vi "UMLEditor Main.vi"(1 "StartProject":string, 3 "StartTarget":string) -> ()   [LabVIEW 2020] (continued)
                        n993 = Unbundle By Name(w2758) -> ("height"=w2757:dbl, "width"=w2754:dbl)
                        n994 = Unbundle By Name(w2751) -> ("Scrolling"=w2732:i32)
                        n995 = Tick Count (ms)() -> (millisecond timer value=w2749:u32)
                        n996 = Equal To 0?(x=w2747) -> (x = 0?=w2746:bool)
                        n997 = Subtract(x=w2749, y=w2747) -> (x-y=w2745:u32)
                        n998 = feedback-in #1(w2732) -> ()
                        n999 = feedback #1(w2732) -> (w2733:i32)
                        n1000 = Select(t=u32 0, s=w2746, f=w2745) -> (s? t:f=w2744:u32)
                        n1001 = Subtract(x=w2732, y=w2733) -> (x-y=w2729:i32)
                        n1002 = Not Equal To 0?(x=w2732) -> (x != 0?=w2731:bool)
                        n1003 = Not Equal To 0?(x=w2729) -> (x != 0?=w2730:bool)
                        n1004 = And(x=w2731, y=w2730) -> ()  [unwired: 1 out]
                        n1005 = case shown="0..750" w2744 {
                          tunnel: w2748 -> [w2764 w2765]
                          tunnel: [w2760 w2765] -> w2740
                          frame Default {
                            n1006 = property on="SearchString" class="Str"("Visible"=FALSE) -> ()  [unwired: 2 in, 2 out]
                            n1007 = local write "SearchString"("" ("SearchString")) -> ()
                            n1008 = Bundle By Name(cluster=w2764, "KeyPressTime"=u32 0) -> (w2760:T5)
                          }
                          frame 0..750 {
                          }
                        }
                        n1009 = case shown="False" FALSE {
                          tunnel: w2757 -> [_ w2910]
                          tunnel: w2756 -> [_ w2909]
                          tunnel: w2740 -> [w2777 w2908]
                          tunnel: [w2776 w2907] -> w2739
                          tunnel: [w2771 w2906] -> w2755
                          tunnel: w2752 -> [w2772 w2905]
                          tunnel: w2754 -> [_ w2904]
                          tunnel: w2750 -> [w2770 w2903]
                          tunnel: w2751 -> [w2779 _]
                          tunnel: w2734 -> [w2778 _]
                          tunnel: w2753 -> [w2775 _]
                          tunnel: w2742 -> [w2774 _]
                          tunnel: w2741 -> [w2773 _]
                          tunnel: [w2769 _] -> w2737
                          tunnel: [w2768 _] -> w2736
                          tunnel: w2735 -> [w2766 _]
                          tunnel: w2729 -> [_ w2901]
                          frame False {
                            n1010 = call <resource>:"UMLEditor_OnHotSpot.vi"("ZoomLevel"=w2766, "ObjectHotspots"=w2773, "Mouse Position"=w2774) -> ("Function"=w2768:T16, "HotSpotCursor"=w2769:bool, "Node"=w2767:refnum<class "AbstractNode.lvclass">)  [unwired: 5 in, 1 out]
                            n1011 = case shown="False" w2769 {
                              tunnel: w2779 -> [w2799 _]
                              tunnel: w2778 -> [w2796 _]
                              tunnel: w2777 -> [w2795 w2887]
                              tunnel: [w2794 w2886] -> w2776
                              tunnel: w2775 -> [w2787 _]
                              tunnel: w2772 -> [w2783 w2889]
                              tunnel: [w2783 w2888] -> w2771
                              tunnel: w2770 -> [_ _]
                              tunnel: w2768 -> [_ w2885]
                              tunnel: w2767 -> [_ w2884]
                              frame False {
                                n1012 = Unbundle By Name(w2799) -> ("Horizontal"=w2798:i32, "Vertical"=w2797:i32)
                                n1013 = property on="Project" class="Ring (strict)"() -> ("Strings []"=w2788:string[])  [unwired: 2 in, 2 out]
                                n1014 = Unbundle By Name(w2796) -> ("button 1"=w2784:bool)
                                n1015 = local read "Project"() -> (w2781:u16)
                                n1016 = Index Array(array=w2788, index=w2781) -> (element=w2782:string)
                                n1017 = Match Pattern(string=w2782, regular expression="^Untitled") -> (offset past match=w2791:i32)  [unwired: 4 out]
                                n1018 = case shown="False" w2784 {
                                tunnel: [_ w2802] -> w2785
                                frame False {
                                }
                                frame True {
                                n1019 = call <resource>:"UMLEditor_GetActiveWindow.vi"() -> ("Project Explorer"=w2802:bool)  [unwired: 1 in, 10 out]
                                }
                                }
                                n1020 = case shown="False" FALSE {
                                tunnel: w2798 -> [w2807 w2829]
                                tunnel: w2797 -> [w2806 w2828]
                                tunnel: w2785 -> [w2805 w2827]
                                tunnel: [w2804 w2826] -> w2793
                                tunnel: w2784 -> [w2803 w2825]
                                frame True {
                                n1021 = while {
                                shift-right: [w2813] -> _
                                shift-left: _ -> [w2812]
                                tunnel: w2807 -> [w2816]
                                tunnel: w2806 -> [w2815]
                                tunnel: w2805 -> [w2813]
                                tunnel: [w2814] -> w2804
                                tunnel: w2803 -> [w2810]
                                stop <- TRUE stop-if-true
                                # "Mouse inside VI"
                                n1022 = property class="VI"() -> ("Front Panel.WinBounds"=w2824:T52, "Front Panel.IsFrontmost"=w2808:bool)  [unwired: 2 in, 2 out]
                                n1023 = Not(x=w2808) -> (.not. x?=w2809:bool)
                                n1024 = Unbundle(w2824) -> ("Left"=w2823:i16, "Top"=w2820:i16, "Right"=w2822:i16, "Bottom"=w2821:i16)
                                n1025 = property on="DragAndDropPath" class="Path"("Visible"=w2809) -> ()  [unwired: 2 in, 2 out]
                                n1026 = In Range and Coerce(upper limit=w2822, x=w2816, lower limit=w2823) -> (In Range?=w2819:bool)  [unwired: 1 out]
                                n1027 = In Range and Coerce(upper limit=w2821, x=w2815, lower limit=w2820) -> (In Range?=w2818:bool)  [unwired: 1 out]
                                n1028 = And(x=w2819, y=w2818) -> (x .and. y?=w2811:bool)
                                n1029 = Compound Arithmetic op=AND(w2811, invert w2810, w2812) -> (w2814:bool)
                                }
                                }
                                frame False {
                                n1030 = while {
                                shift-right: [w2833] -> _
                                shift-left: _ -> [w2832]
                                tunnel: w2829 -> [w2836]
                                tunnel: w2828 -> [w2835]
                                tunnel: w2827 -> [w2833]
                                tunnel: [w2834] -> w2826
                                tunnel: w2825 -> [w2830]
                                stop <- TRUE stop-if-true
                                # "Mouse inside VI"
                                n1031 = property class="VI" props=["Front Panel.WinBounds", "Front Panel.IsFrontmost"]() -> ("Front Panel.WinBounds"=w2844:T52)  [unwired: 2 in, 3 out]
                                n1032 = Unbundle(w2844) -> ("Left"=w2843:i16, "Top"=w2840:i16, "Right"=w2842:i16, "Bottom"=w2841:i16)
                                n1033 = In Range and Coerce(upper limit=w2842, x=w2836, lower limit=w2843) -> (In Range?=w2839:bool)  [unwired: 1 out]
                                n1034 = In Range and Coerce(upper limit=w2841, x=w2835, lower limit=w2840) -> (In Range?=w2838:bool)  [unwired: 1 out]
                                n1035 = And(x=w2839, y=w2838) -> (x .and. y?=w2831:bool)
                                n1036 = Compound Arithmetic op=AND(w2831, invert w2830, w2832) -> (w2834:bool)
                                }
                                }
                                }
                                n1037 = while {
                                shift-right: [w2880] -> w2801
                                shift-left: _ -> [w2882]
                                stop <- TRUE stop-if-true
                                n1038 = Increment(x=w2882) -> (x+1=w2881:u8)
                                n1039 = To Unsigned Byte Integer(number=w2881) -> (unsigned 8bit integer=w2880:u8)
                                }
                                n1040 = Empty String/Path?(string/path=w2782) -> (empty?=w2800:bool)
                                n1041 = Greater Or Equal To 0?(x=w2791) -> (x >= 0?=w2790:bool)
                                n1042 = call <resource>:"UMLEditor_SetMouseCursor.vi"("error in (no error)"=w2783, "CursorType"=UMLEditor_Cursortype."Arrow") -> ()  [unwired: 8 in, 2 out]
                                n1043 = Or(x=w2800, y=w2790) -> (x .or. y?=w2789:bool)
                                n1044 = case shown="0" w2801 {
                                tunnel: w2789 -> [w2851 _ _ _]
                                tunnel: w2782 -> [w2850 _ _ _]
                                tunnel: w2787 -> [_ _ _ _]
                                tunnel: w2781 -> [w2849 _ _ _]
                                frame 0 {
                                n1045 = case shown="True" w2851 {
                                tunnel: w2850 -> [_ _]
                                tunnel: w2849 -> [_ w2855]
                                frame False {
                                }
                                frame True {
                                n1046 = call <resource>:"GDSProject_GetProjects.vi"("OpenProjectRef(True)"=FALSE) -> ("Projects"=w2858:string[], "error out"=w2861:errorcluster)  [unwired: 2 in, 15 out]
                                n1047 = Array Size(array=w2858) -> (size(s)=w2857:i32)
                                n1048 = Empty Array?(array=w2858) -> (empty?=w2862:bool)
                                n1049 = Decrement(x=w2857) -> (x-1=w2856:i32)
                                n1050 = Max & Min(x=w2856, y=w2855) -> (min(x,y)=w2854:i32)  [unwired: 1 out]
                                n1051 = Max & Min(x=w2854, y=0) -> (max(x,y)=w2852:i32)  [unwired: 1 out]
                                n1052 = Index Array(array=w2858, index=w2852) -> (element=w2860:string)
                                n1053 = property on="Project" class="Ring (strict)"("Strings []"=w2858, "Value"=w2852) -> ()  [unwired: 2 in, 2 out]
                                n1054 = case shown="False" w2862 {
                                tunnel: w2860 -> [w2868 _]
                                tunnel: w2861 -> [w2869 w2879]
                                tunnel: [w2866 w2878] -> _
                                frame False {
                                n1055 = call <resource>:"GetRelativePathOption.vi"() -> ("UseProjectFolderAsBasePath"=w2871:bool)  [unwired: 1 in, 18 out]
                                n1056 = call <resource>:"UMLEditor_TargetDialog.vi"("error in (no error)"=w2869, "Target"="My Computer" ("element"), "GetProjectRefByName"=w2868) -> ("error out"=w2866:errorcluster, "ProjectFolder"=w2867:path, "TargetIndex"=w2864:u16, "Targets"=w2865:string[])  [unwired: 4 in, 1 out]
                                n1057 = case shown="True" w2871 {
                                tunnel: w2867 -> [_ w2873]
                                tunnel: File_StoredPathesActions."Set Path" ("Method (Get Path)") -> [_ w2872]
                                frame False {
                                }
                                frame True {
                                n1058 = call <resource>:"File_ApplicationPaths.vi"("PathName"=UMLEditor_StoredPathes."ClassBasePath" ("UMLPathes"), "Path In"=w2873, "Method (Get Path)"=w2872) -> ()  [unwired: 1 in, 16 out]
                                }
                                }
                                n1059 = property on="Target" class="Ring (strict)"("Strings []"=w2865, "Value"=w2864) -> ()  [unwired: 2 in, 2 out]
                                }
                                frame True {
                                n1060 = call <resource>:"CommonVIs_UmlOpenVIRef.vi"("ProjectNameIn"="clear", "error in"=w2879) -> ("error out"=w2878:errorcluster)  [unwired: 2 in, 7 out]
                                n1061 = property on="Target" class="Ring (strict)"("Strings []"=string[] [], "Value"=u16 0 ("icon")) -> ()  [unwired: 2 in, 2 out]
                                }
                                }
                                }
                                }
                                }
                                frame 1 {
                                }
                                frame 2 {
                                }
                                frame Default {
                                }
                                }
                                n1062 = case shown="False" w2793 {
                                tunnel: w2795 -> [w2845 w2848]
                                tunnel: [w2845 w2847] -> w2794
                                frame False {
                                }
                                frame True {
                                n1063 = Bundle By Name(cluster=w2848, "state"=UMLEditor_statesType."AddNodeFromProjectTree") -> (w2847:T5)
                                }
                                }
                              }
                              frame True {
                                n1064 = case shown="Default" w2885 {
                                tunnel: w2889 -> [w2892 w2898]
                                tunnel: [w2890 w2899] -> w2888
                                tunnel: w2885 -> [w2893 _]
                                frame Default {
                                n1065 = case shown="\"SE\", \"NW\"" w2893 {
                                tunnel: [_ UMLEditor_Cursortype."NS" ("CursorType") UMLEditor_Cursortype."NESW" ("CursorType") UMLEditor_Cursortype."WE" ("CursorType") UMLEditor_Cursortype."NWSE" ("CursorType")] -> w2891
                                frame Default {
                                }
                                frame "N", "S" {
                                }
                                frame "NE", "SW" {
                                }
                                frame "E", "W" {
                                }
                                frame "SE", "NW" {
                                }
                                }
                                n1066 = call <resource>:"UMLEditor_SetMouseCursor.vi"("error in (no error)"=w2892, "CursorType"=w2891) -> ("error out"=w2890:errorcluster)  [unwired: 8 in, 1 out]
                                }
                                frame "Expand", "Collaps" {
                                n1067 = call <resource>:"UMLEditor_SetMouseCursor.vi"("error in (no error)"=w2898, "CursorType"=UMLEditor_Cursortype."Finger") -> ("error out"=w2899:errorcluster)  [unwired: 8 in, 1 out]
                                }
                                }
                                n1068 = Bundle By Name(cluster=w2887, "HotSpotNode"=w2884) -> (w2886:T5)
                              }
                            }
                          }
                          frame True {
                            n1069 = property class="VI"() -> ("Front Panel.IsFrontmost"=w2902:bool)  [unwired: 2 in, 2 out]
                            n1070 = case shown="True" w2902 {
                              tunnel: w2901 -> [_ w2921]
                              tunnel: w2910 -> [_ w2920]
                              tunnel: w2909 -> [_ w2919]
                              tunnel: w2908 -> [w2912 w2918]
                              tunnel: [w2912 w2917] -> w2907
                              tunnel: [w2911 w2916] -> w2906
                              tunnel: w2905 -> [w2911 w2915]
                              tunnel: w2904 -> [_ w2914]
                              tunnel: w2903 -> [_ w2913]
                              frame False {
                              }
                              frame True {
                                n1071 = case shown="False" w2919 {
                                tunnel: w2921 -> [w2922 w2957]
                                tunnel: w2920 -> [w2950 _]
                                tunnel: w2918 -> [w2932 w2960]
                                tunnel: [w2932 w2961] -> w2917
                                tunnel: [w2944 w2959] -> w2916
                                tunnel: w2915 -> [w2944 w2958]
                                tunnel: w2914 -> [w2928 _]
                                tunnel: w2913 -> [_ _]
                                frame False {
                                w2936 = 0 ("lower limit")
                                n1072 = Unbundle By Name(w2932) -> ("zoom"=w2929:dbl)
                                n1073 = Multiply(x=w2929, y=w2950) -> (x*y=w2931:dbl)
                                n1074 = Multiply(x=w2929, y=w2928) -> (x*y=w2930:dbl)
                                n1075 = In Range and Coerce(upper limit=10, x=w2922, lower limit=-10) -> ()  [unwired: 2 out]
                                n1076 = property on="Picture" class="Pict"() -> ("Draw Area Size"=w2953:T42)  [unwired: 2 in, 2 out]
                                n1077 = To Long Integer(number=w2930) -> (32bit integer=w2940:i32)
                                n1078 = To Long Integer(number=w2931) -> (32bit integer=w2947:i32)
                                n1079 = property on="Picture" class="Pict"() -> ("Origin:Top"=w2926:i16, "Origin:Left"=w2935:i16)  [unwired: 2 in, 2 out]
                                n1080 = Unbundle By Name(w2953) -> ("Height"=w2949:u32, "Width"=w2941:u32)
                                n1081 = Subtract(x=w2926, y=w2922) -> (x-y=w2952:i32)
                                n1082 = Subtract(x=w2935, y=w2922) -> (x-y=w2934:i32)
                                n1083 = To Long Integer(number=w2941) -> (32bit integer=w2939:i32)
                                n1084 = Subtract(x=w2940, y=w2939) -> (x-y=w2938:i32)
                                n1085 = Max & Min(x=w2938, y=w2936) -> (max(x,y)=w2937:i32)  [unwired: 1 out]
                                n1086 = In Range and Coerce(upper limit=w2937, x=w2934, lower limit=w2936) -> (coerced(x)=w2933:i32)  [unwired: 1 out]
                                n1087 = To Long Integer(number=w2949) -> (32bit integer=w2942:i32)
                                n1088 = Subtract(x=w2947, y=w2942) -> (x-y=w2948:i32)
                                n1089 = Max & Min(x=w2948, y=0 ("lower limit")) -> (max(x,y)=w2945:i32)  [unwired: 1 out]
                                n1090 = In Range and Coerce(upper limit=w2945, x=w2952, lower limit=0) -> (coerced(x)=w2927:i32)  [unwired: 1 out]
                                n1091 = Not Equal?(x=w2927, y=w2926) -> (x != y?=w2925:bool)
                                n1092 = Select(t=w2935, s=w2925, f=w2933) -> (s? t:f=w2943:i32)
                                n1093 = property on="Picture" class="Pict"("Origin:Top"=w2927, "Origin:Left"=w2943) -> ()  [unwired: 2 in, 2 out]
                                }
                                frame True {
                                w2962 = 1.5 ("x")
                                n1094 = Unbundle By Name(w2960) -> ("graphics"=w2969:refnum<class "Graphics.lvclass">, "zoom"=w2955:dbl)
                                n1095 = Less Than 0?(x=w2957) -> (x < 0?=w2967:bool)
                                n1096 = Not(x=w2967) -> (.not. x?=w2954:bool)
                                n1097 = Multiply(x=w2955, y=w2962) -> (x*y=w2968:dbl)
                                n1098 = Divide(x=w2955, y=w2962) -> (x/y=w2966:dbl)
                                n1099 = Select(t=w2968, s=w2954, f=w2966) -> (s? t:f=w2965:dbl)
                                n1100 = In Range and Coerce(upper limit=5.0625, x=w2965, lower limit=0.197530864) -> (coerced(x)=w2956:dbl)  [unwired: 1 out]
                                n1101 = call <resource>:"scale.vi"("reference"=w2969, "scaleX"=w2956, "scaleY"=w2956, "error in (no error)"=w2958) -> ("error out"=w2959:errorcluster)  [unwired: 15 out]
                                n1102 = Bundle By Name(cluster=w2960, "zoom"=w2956, "state"=UMLEditor_statesType."Repaint") -> (w2961:T5)
                                }
                                }
                              }
                            }
                          }
                        }
                        n1103 = Bundle By Name(cluster=w2739, "HotSpotCursor"=w2737, "HotSpotFunction"=w2736) -> (w2738:T5)
                      }
                      frame True {
                        n1104 = disable-structure shown="Disabled" {
                          frame Disabled {
                            n1105 = property class="VI"() -> ("Front Panel Window:Panel Bounds"=w2987:T52)  [unwired: 2 in, 2 out]
                            n1106 = Unbundle By Name(w2987) -> ("Left"=w2981:i16, "Top"=w2978:i16, "Right"=w2982:i16, "Bottom"=w2979:i16)
                            n1107 = Subtract(x=w2979, y=w2978) -> (x-y=w2977:i16)
                            n1108 = Subtract(x=w2982, y=w2981) -> (x-y=w2980:i16)
                            n1109 = Subtract(x=w2980, y=23 ("X")) -> (x-y=w2986:i32)
                            n1110 = Subtract(x=w2977, y=100) -> (x-y=w2985:i32)
                            n1111 = Bundle(w2986, w2985) -> (w2976:cluster{i32, i32})  [unwired: 1 in]
                            n1112 = property on="Picture" class="Pict"("Draw Area Size"=w2976) -> ()  [unwired: 2 in, 2 out]
                          }
                          frame Enabled {
                          }
                        }
                        n1113 = Bundle By Name(cluster=w2975, "state"=UMLEditor_statesType."Repaint", "ResizePanelInProgress"=FALSE) -> (w2973:T5)
                      }
                    }
                  }
                  frame True {
                    n1114 = property on="Picture" class="Pict"() -> ("Mouse"=w2992:T41)  [unwired: 2 in, 2 out]
                    n1115 = Unbundle By Name(w2992) -> ("Mouse Position"=w2991:cluster{"X":i32, "Y":i32})
                    n1116 = Unbundle By Name(w2990) -> ("zoom"=w2999:dbl, "offset"=w2997:T9)
                    n1117 = Add(x=w2997, y=w2991) -> (x+y=w2998:T9)
                    n1118 = Divide(x=w2998, y=w2999) -> (x/y=w2995:T9)
                    n1119 = call-dynamic "findNode.vi"("reference"=w2988, "point2D"=w2995, "error in (no error)"=w2989) -> ("node"=w2996:refnum<class "AbstractNode.lvclass">, "found"=w2993:bool, "error out"=w2994:errorcluster)  [unwired: 13 in, 1 out]
                    n1120 = case shown="True" w2993 {
                      tunnel: [w3001 w3004] -> w3000
                      tunnel: w2996 -> [_ w3008]
                      tunnel: w2995 -> [_ w3007]
                      tunnel: w2994 -> [w3001 w3006]
                      frame False {
                      }
                      frame True {
                        n1121 = call-dynamic "GetContextHelpInfo.vi"("reference"=w3008, "MousePos"=w3007, "error in (no error)"=w3006) -> ("ContextHelpInfoExist"=w3002:bool, "ContextHelpInfo"=w3003:variant, "error out"=w3005:errorcluster)  [unwired: 13 in, 1 out]
                        n1122 = case shown="True" w3002 {
                          tunnel: w3005 -> [w3009 w3012]
                          tunnel: [w3009 w3011] -> w3004
                          tunnel: w3003 -> [_ w3010]
                          frame False {
                          }
                          frame True {
                            n1123 = call <resource>:"ContextHelp_SendMessageToPopUp.vi"("PopUpMessage"=w3010, "error in (no error)"=w3012) -> ("error out"=w3011:errorcluster)  [unwired: 1 in, 16 out]
                          }
                        }
                      }
                    }
                  }
                }
              }
              frame True {
                (unwired) UMLEditor_HotSpotType."Expand" ("HotSpotFunction")
                n1124 = Unbundle By Name(w3017) -> ("graphics"=w3041:refnum<class "Graphics.lvclass">, "rubberBandStart"=w3040:T9, "dragStartPoint"=w3024:T9, "dragStartBounds"=w3032:T10, "selected"=w3023:T7, "lastMousePoint"=w3013:T9)
                n1125 = Unbundle By Name(w3017) -> ("HotSpotCursor"=w3020:bool, "HotSpotFunction"=w3022:T16)
                n1126 = Unbundle By Name(w3017) -> ("ShiftDown"=w3016:bool, "CtrlDown"=w3015:bool)
                n1127 = Unbundle By Name(w3017) -> ("selected"=w3034:T7, "SelectedNodes"=w3033:refnum<class "AbstractNode.lvclass">[], "selectedEdge"=w3025:refnum<class "AbstractEdge.lvclass">)
                n1128 = property on="Picture" class="Pict"() -> ("Mouse"=w3018:T41)  [unwired: 2 in, 2 out]
                n1129 = Unbundle By Name(w3018) -> ("Mouse Position.X"=w3045:i32, "Mouse Position.Y"=w3044:i32, "Mouse Position"=w3027:cluster{"X":i32, "Y":i32})
                n1130 = Unbundle By Name(w3017) -> ("offset"=w3026:T9, "zoom"=w3037:dbl)
                n1131 = Add(x=w3027, y=w3026) -> (x+y=w3028:T9)
                n1132 = Add(x=w3045, y=w3044) -> (x+y=w3043:i32)
                n1133 = Divide(x=w3028, y=w3037) -> (x/y=w3029:T9)
                n1134 = Equal?(x=w3013, y=w3029) -> (x = y?=w3030:bool)
                n1135 = call <resource>:"Point getValues.vi"("point2D"=w3040) -> ("valid"=w3039:bool)  [unwired: 18 out]
                n1136 = call <resource>:"Point getValues.vi"("point2D"=w3024) -> ("valid"=w3038:bool)  [unwired: 18 out]
                n1137 = Less Than 0?(x=w3043) -> (x < 0?=w3031:bool)
                n1138 = Or(x=w3030, y=w3031) -> (x .or. y?=w3021:bool)
                n1139 = Compound Arithmetic op=AND(w3021, invert w3020) -> (w3019:bool)
                n1140 = case shown="False" w3019 {
                  tunnel: w3029 -> [w3067 _]
                  tunnel: w3041 -> [w3066 _]
                  tunnel: w3017 -> [w3054 w3285]
                  tunnel: [w3053 w3284] -> w3042
                  tunnel: w3040 -> [w3065 _]
                  tunnel: w3039 -> [w3064 _]
                  tunnel: w3038 -> [w3063 _]
                  tunnel: w3035 -> [w3062 w3283]
                  tunnel: [w3061 w3283] -> w3036
                  tunnel: w3017 -> [w3060 _]
                  tunnel: w3034 -> [w3059 _]
                  tunnel: w3033 -> [w3058 _]
                  tunnel: w3032 -> [w3057 _]
                  tunnel: w3024 -> [w3056 _]
                  tunnel: w3014 -> [w3055 _]
                  tunnel: w3030 -> [_ w3282]
                  tunnel: w3025 -> [w3052 _]
                  tunnel: w3023 -> [w3051 _]
                  tunnel: w3013 -> [w3050 _]
                  tunnel: w3014 -> [w3049 _]
                  tunnel: w3020 -> [w3048 _]
                  tunnel: w3022 -> [w3047 _]
                  tunnel: w3016 -> [_ _]
                  tunnel: w3015 -> [_ _]
                  tunnel: w3015 -> [w3046 _]
                  frame False {
                    n1141 = case shown="False" w3064 {
                      tunnel: w3067 -> [w3078 w3248]
                      tunnel: w3066 -> [_ w3255]
                      tunnel: w3065 -> [_ w3249]
                      tunnel: w3063 -> [w3085 _]
                      tunnel: w3062 -> [w3083 w3254]
                      tunnel: [w3084 w3253] -> w3061
                      tunnel: w3060 -> [w3082 _]
                      tunnel: w3059 -> [w3081 _]
                      tunnel: w3058 -> [w3080 _]
                      tunnel: w3057 -> [w3079 _]
                      tunnel: w3056 -> [w3077 _]
                      tunnel: w3055 -> [w3076 _]
                      tunnel: w3054 -> [w3075 w3252]
                      tunnel: [w3074 w3251] -> w3053
                      tunnel: w3052 -> [w3073 _]
                      tunnel: w3051 -> [_ w3250]
                      tunnel: w3050 -> [w3072 _]
                      tunnel: w3049 -> [w3071 _]
                      tunnel: w3048 -> [w3070 _]
                      tunnel: w3047 -> [w3069 _]
                      tunnel: w3046 -> [w3068 _]
                      frame False {
                        n1142 = case shown="True" w3085 {
                          tunnel: [w3087 w3101] -> w3084
                          tunnel: w3083 -> [w3087 w3102]
                          tunnel: w3082 -> [_ _]
                          tunnel: w3081 -> [_ w3103]
                          tunnel: w3080 -> [_ w3100]
                          tunnel: w3079 -> [_ w3093]
                          tunnel: w3078 -> [_ w3099]
                          tunnel: w3077 -> [_ w3098]
                          tunnel: w3076 -> [_ w3097]
                          tunnel: w3075 -> [w3086 w3096]
                          tunnel: [w3086 w3095] -> w3074
                          tunnel: w3073 -> [_ w3094]
                          tunnel: w3072 -> [_ w3092]
                          tunnel: w3071 -> [_ w3091]
                          tunnel: w3070 -> [_ w3090]
                          tunnel: w3069 -> [_ w3089]
                          tunnel: w3068 -> [_ w3088]
                          frame False {
                          }
                          frame True {
                            n1143 = case shown="\"Edge\"" w3103 {
                              tunnel: w3102 -> [w3105 w3112 w3230]
                              tunnel: [w3105 w3116 w3238] -> w3101
                              tunnel: w3100 -> [_ w3110 w3229]
                              tunnel: w3099 -> [_ w3113 w3228]
                              tunnel: w3098 -> [_ _ w3243]
                              tunnel: w3097 -> [_ _ _]
                              tunnel: w3096 -> [w3104 w3118 w3240]
                              tunnel: [w3104 w3114 w3236] -> w3095
                              tunnel: w3094 -> [_ _ w3235]
                              tunnel: w3093 -> [_ _ _]
                              tunnel: w3092 -> [_ w3111 _]
                              tunnel: w3091 -> [_ w3109 _]
                              tunnel: w3090 -> [_ w3108 _]
                              tunnel: w3089 -> [_ w3107 _]
                              tunnel: w3088 -> [_ w3106 _]
                              frame Default {
                              }
                              frame "Node" {
                                n1144 = Bundle By Name(cluster=w3118, "state"=UMLEditor_statesType."Repaint", "lastMousePoint"=w3113) -> (w3115:T5)
                                n1145 = case shown="False" w3108 {
                                tunnel: [w3126 w3182] -> w3116
                                tunnel: w3115 -> [w3125 w3178]
                                tunnel: [w3124 w3177] -> w3114
                                tunnel: w3113 -> [w3123 w3186]
                                tunnel: w3112 -> [w3122 w3183]
                                tunnel: w3111 -> [w3121 w3185]
                                tunnel: w3110 -> [w3120 w3181]
                                tunnel: w3109 -> [_ _]
                                tunnel: w3107 -> [_ w3184]
                                tunnel: w3106 -> [w3119 _]
                                frame False {
                                n1146 = case shown="False" w3119 {
                                tunnel: [w3136 w3172] -> w3126
                                tunnel: w3125 -> [w3135 w3176]
                                tunnel: [w3134 w3173] -> w3124
                                tunnel: w3123 -> [w3133 _]
                                tunnel: w3122 -> [w3132 w3172]
                                tunnel: w3121 -> [w3131 _]
                                tunnel: w3120 -> [w3130 _]
                                frame False {
                                n1147 = for {
                                tunnel: w3130 -> [w3139] mode=indexing
                                shift-right: [w3140] -> w3129
                                shift-left: refnum<class "AbstractNode.lvclass">[] [] -> [w3141]
                                n1148 = call <resource>:"GetAllChildrenRecursive.vi"("reference"=w3139) -> ("children"=w3138:refnum<class "AbstractNode.lvclass">[])  [unwired: 1 in, 17 out]
                                n1149 = Build Array (concatenate)(w3141, w3138) -> (w3140:refnum<class "AbstractNode.lvclass">[])
                                }
                                n1150 = for {
                                tunnel: w3130 -> [w3165] mode=indexing
                                tunnel: w3133 -> [w3161]
                                shift-right: [w3163] -> w3128
                                shift-left: w3132 -> [w3164]
                                tunnel: w3131 -> [w3160]
                                tunnel: w3129 -> [w3147]
                                w3150 = 0.0 ("t")
                                n1151 = Subtract(x=w3161, y=w3160) -> (x-y=w3162:T9)
                                n1152 = call-dynamic "getBounds.vi"("reference"=w3165, "error in (no error)"=w3164) -> ("reference out"=w3144:refnum<class "AbstractNode.lvclass">, "bounds"=w3159:T10, "error out"=w3145:errorcluster)  [unwired: 15 in]
                                n1153 = Unbundle(w3159) -> ("x"=w3158:dbl, "y"=w3152:dbl)  [unwired: 2 out]
                                n1154 = Unbundle(w3162) -> ("x"=w3151:dbl, "y"=w3149:dbl)
                                n1155 = call-dynamic "getParent.vi"("reference"=w3144, "error in (no error)"=w3145) -> ("reference out"=w3142:refnum<class "AbstractNode.lvclass">, "error out"=w3143:errorcluster)  [unwired: 13 in, 3 out]
                                n1156 = Search 1D Array(1D array=w3147, element=w3144) -> (index of element=w3146:i32)  [unwired: 1 out]
                                n1157 = Add(x=w3158, y=w3151) -> (x+y=w3157:dbl)
                                n1158 = Add(x=w3152, y=w3149) -> (x+y=w3153:dbl)
                                n1159 = Less Than 0?(x=w3157) -> (x < 0?=w3156:bool)
                                n1160 = Less Than 0?(x=w3153) -> (x < 0?=w3154:bool)
                                n1161 = Select(t=w3150, s=w3156, f=w3151) -> (s? t:f=w3155:dbl)
                                n1162 = Select(t=w3150, s=w3154, f=w3149) -> (s? t:f=w3148:dbl)
                                n1163 = case shown="-1" w3146 {
                                tunnel: w3143 -> [w3166 w3171]
                                tunnel: [w3166 w3170] -> w3163
                                tunnel: w3155 -> [_ w3169]
                                tunnel: w3148 -> [_ w3168]
                                tunnel: w3142 -> [_ w3167]
                                frame 0, Default {
                                }
                                frame -1 {
                                n1164 = call-dynamic "translate.vi"("reference"=w3167, "dx"=w3169, "dy"=w3168, "error in (no error)"=w3171) -> ("error out"=w3170:errorcluster)  [unwired: 14 in, 1 out]
                                }
                                }
                                }
                                n1165 = call <resource>:"UMLEditor setDiagramInfo.vi"("error in (no error)"=w3128, "localVariablesIn"=w3135, "action"=enum16{"Name/Dir", "Unsaved", "Saved"}."Unsaved") -> ("localVariablesOut"=w3134:T5, "error out"=w3136:errorcluster)  [unwired: 2 in, 13 out]
                                }
                                frame True {
                                n1166 = Bundle By Name(cluster=w3176, "state"=UMLEditor_statesType."CopyPaste", "CtrlDown"=FALSE) -> (w3173:T5)
                                }
                                }
                                }
                                frame True {
                                n1167 = Subtract(x=w3186, y=w3185) -> (x-y=w3187:T9)
                                n1168 = Unbundle(w3187) -> ("x"=w3180:dbl, "y"=w3179:dbl)
                                n1169 = case shown="Default" w3184 {
                                selector: w3184 -> [_ w3195 w3212]
                                tunnel: w3183 -> [w3189 w3194 w3217]
                                tunnel: [w3189 w3192 w3216] -> w3182
                                tunnel: w3181 -> [_ w3193 w3215]
                                tunnel: w3180 -> [_ _ w3214]
                                tunnel: w3179 -> [_ _ w3213]
                                tunnel: w3178 -> [w3188 w3191 w3211]
                                tunnel: [w3188 w3190 w3211] -> w3177
                                frame Default {
                                }
                                frame "Expand", "Collaps" {
                                n1170 = disable-structure shown="Disabled" {
                                disable-tunnel: w3195 -> [w3208 _]
                                disable-tunnel: w3194 -> [w3205 w3209]
                                disable-tunnel: w3193 -> [w3204 _]
                                disable-tunnel: [w3200 w3209] -> w3192
                                disable-tunnel: w3191 -> [w3199 w3210]
                                disable-tunnel: [w3196 w3210] -> w3190
                                frame Disabled {
                                n1171 = Index Array(array=w3204) -> (element=w3203:refnum<class "AbstractNode.lvclass">)  [unwired: 1 in]
                                n1172 = Equal?(x=w3208, y=UMLEditor_HotSpotType."Collaps") -> (x = y?=w3206:bool)
                                n1173 = call-dynamic "Collaps.vi"("reference in"=w3203, "Collaps"=w3206, "error in (no error)"=w3205) -> ("error out"=w3201:errorcluster)  [unwired: 15 in, 1 out]
                                n1174 = Bundle By Name(cluster=w3199, "HotSpotCursor"=FALSE) -> (w3197:T5)
                                n1175 = call <resource>:"UMLEditor setDiagramInfo.vi"("error in (no error)"=w3201, "localVariablesIn"=w3197, "action"=enum16{"Name/Dir", "Unsaved", "Saved"}."Unsaved") -> ("localVariablesOut"=w3196:T5, "error out"=w3200:errorcluster)  [unwired: 2 in, 13 out]
                                }
                                frame Enabled {
                                }
                                }
                                }
                                frame "N".."NW" {
                                n1176 = for {
                                shift-right: [w3222] -> w3216
                                shift-left: w3217 -> [w3223]
                                tunnel: w3215 -> [w3221] mode=indexing
                                tunnel: w3214 -> [w3220]
                                tunnel: w3213 -> [w3219]
                                tunnel: w3212 -> [w3218]
                                n1177 = call-dynamic "Resize.vi"("reference in"=w3221, "dx"=w3220, "dy"=w3219, "Positions"=w3218, "error in (no error)"=w3223) -> ("error out"=w3222:errorcluster)  [unwired: 13 in, 1 out]
                                }
                                }
                                }
                                }
                                }
                              }
                              frame "Edge" {
                                n1178 = Array Size(array=w3229) -> (size(s)=w3224:i32)
                                n1179 = Unbundle By Name(w3243) -> ("x"=w3242:dbl, "y"=w3241:dbl)
                                n1180 = case shown="2" w3224 {
                                tunnel: w3229 -> [_ w3247]
                                tunnel: [w3245 w3246] -> w3225
                                frame 2 {
                                n1181 = call <resource>:"GetObject.vi"("RefNum"=-1 ("type")) -> ("reference"=w3245:refnum<class "AbstractNode.lvclass">)  [unwired: 17 in, 1 out]
                                }
                                frame Default {
                                n1182 = Index Array(array=w3247) -> (element=w3246:refnum<class "AbstractNode.lvclass">)  [unwired: 1 in]
                                }
                                }
                                n1183 = Unbundle(w3228) -> ("x"=w3232:dbl, "y"=w3231:dbl)
                                n1184 = Subtract(x=w3232, y=w3242) -> (x-y=w3234:dbl)
                                n1185 = Subtract(x=w3231, y=w3241) -> (x-y=w3233:dbl)
                                n1186 = Bundle By Name(cluster=w3240, "state"=UMLEditor_statesType."Repaint", "lastMousePoint"=w3228, "dragStartPoint"=w3228) -> (w3237:T5)
                                n1187 = call-dynamic "Translate.vi"("reference"=w3235, "dx"=w3234, "dy"=w3233, "StartEndNode"=w3225, "error in (no error)"=w3230) -> ("error out"=w3226:errorcluster)  [unwired: 13 in, 1 out]
                                n1188 = call <resource>:"UMLEditor setDiagramInfo.vi"("error in (no error)"=w3226, "localVariablesIn"=w3237, "action"=enum16{"Name/Dir", "Unsaved", "Saved"}."Unsaved") -> ("localVariablesOut"=w3236:T5, "error out"=w3238:errorcluster)  [unwired: 2 in, 13 out]
                              }
                            }
                          }
                        }
                      }
                      frame True {
                        n1189 = case shown="\"None\"" w3250 {
                          tunnel: w3255 -> [w3272 w3281]
                          tunnel: w3254 -> [w3274 w3280]
                          tunnel: [w3273 w3279] -> w3253
                          tunnel: w3249 -> [w3267 w3277]
                          tunnel: w3248 -> [w3266 w3276]
                          frame "None" {
                            n1190 = Unbundle(w3267) -> ("x"=w3265:dbl, "y"=w3261:dbl)
                            n1191 = Unbundle(w3266) -> ("x"=w3264:dbl, "y"=w3260:dbl)
                            n1192 = Max & Min(x=w3265, y=w3264) -> (max(x,y)=w3263:dbl, min(x,y)=w3262:dbl)
                            n1193 = Max & Min(x=w3261, y=w3260) -> (max(x,y)=w3259:dbl, min(x,y)=w3258:dbl)
                            n1194 = Subtract(x=w3263, y=w3262) -> (x-y=w3269:dbl)
                            n1195 = Subtract(x=w3259, y=w3258) -> (x-y=w3268:dbl)
                            n1196 = Bundle By Name(cluster=T10 {"x"=0.0, "y"=0.0, "width"=0.0, "height"=0.0} ("rectangle"), "x"=w3262, "y"=w3258, "width"=w3269, "height"=w3268) -> (w3257:T10)
                            n1197 = call <resource>:"drawTempRectangle.vi"("reference"=w3272, "rectangle"=w3257, "color(if not used=default color)"=u32 16711680, "error in (no error)"=w3274) -> ("picture"=w3256:picture, "error out"=w3273:errorcluster)  [unwired: 4 in, 10 out]
                            n1198 = local write "Picture"(w3256) -> ()
                          }
                          frame Default {
                            n1199 = Build Array(w3277, w3276) -> (w3278:T9[])
                            n1200 = call-dynamic "drawTempLine.vi"("reference"=w3281, "points"=w3278, "error in (no error)"=w3280) -> ("new picture"=w3275:picture, "error out"=w3279:errorcluster)  [unwired: 14 in, 1 out]
                            n1201 = local write "Picture"(w3275) -> ()
                          }
                        }
                        n1202 = Bundle By Name(cluster=w3252, "lastMousePoint"=w3248) -> (w3251:T5)
                      }
                    }
                  }
                  frame True {
                    n1203 = case shown="False" w3282 {
                      tunnel: w3285 -> [w3289 w3291]
                      tunnel: [w3288 w3291] -> w3284
                      frame False {
                        w3287 = T9 {"x"=nan, "y"=nan} ("rubberBandStart")
                        n1204 = Bundle By Name(cluster=w3289, "butDwn"=FALSE ("b_dwn"), "rubberBandStart"=w3287, "dragStartPoint"=w3287, "dragStartBounds"=T10 {"x"=nan, "y"=nan, "width"=nan, "height"=nan}) -> (w3288:T5)
                      }
                      frame True {
                      }
                    }
                  }
                }
              }
            }
          }
        }
        n1205 = Unbundle By Name(w262) -> ("butDwn"=w248:bool, "Sync"=w251:bool, "state"=w250:T6)
        n1206 = Equal?(x=w250, y=UMLEditor_statesType."Idle") -> (x = y?=w252:bool)
        n1207 = Compound Arithmetic op=AND(invert w248, w251, w252) -> (w249:bool)
        n1208 = Select(t=UMLEditor_statesType."AutoSync" ("state"), s=w249, f=w250) -> (s? t:f=w255:T6)
      }
      frame "AutoSync" {
        (unwired) UMLEditor_statesType."Idle" ("state")
        # "Have we been idle for a while?\nIf so, do a sync"
        n1209 = Unbundle By Name(w3295) -> ("LastSync"=w3302:timestamp, "SyncTime"=w3301:u32, "ForceSyncNow"=w3303:bool)
        n1210 = Get Date/Time In Seconds() -> (seconds since 1Jan1904=w3293:timestamp)
        n1211 = Subtract(x=w3293, y=w3302) -> (x-y=w3300:dbl)
        n1212 = Subtract(x=w3301, y=w3300) -> (x-y=w3299:dbl)
        n1213 = To Long Integer(number=w3299) -> (32bit integer=w3296:i32)
        n1214 = Max & Min(x=0, y=w3296) -> (max(x,y)=w3292:i32)  [unwired: 1 out]
        n1215 = Equal To 0?(x=w3292) -> (x = 0?=w3297:bool)
        n1216 = Or(x=w3297, y=w3303) -> (x .or. y?=w3304:bool)
        n1217 = case shown="True" w3304 {
          tunnel: w3310 -> [_ _]
          tunnel: w3295 -> [_ w3341]
          tunnel: [_ w3325] -> w3309
          tunnel: w3303 -> [_ w3326]
          tunnel: w3292 -> [w3313 _]
          tunnel: w3295 -> [w3312 w3324]
          tunnel: [w3312 w3323] -> w3294
          tunnel: w3293 -> [_ w3322]
          frame False {
            n1218 = feedback-in #2(w3313) -> ()
            n1219 = feedback #2() -> (w3315:i32)  [unwired: 1 in]
            n1220 = Not Equal?(x=w3315, y=w3313) -> (x != y?=w3314:bool)
            n1221 = case shown="True" w3314 {
              tunnel: w3313 -> [_ w3316]
              frame False {
              }
              frame True {
                n1222 = case shown="Default" w3316 {
                  selector: w3316 -> [_ w3319]
                  tunnel: ["Auto sync in 1 second" ("format string") w3320] -> w3317
                  frame 1 {
                  }
                  frame Default {
                    n1223 = Format Into String(format string="Auto sync in %d seconds", w3319) -> (resulting string=w3320:string)  [unwired: 2 in, 1 out]
                  }
                }
                n1224 = local write "StatusBar"(w3317) -> ()
              }
            }
          }
          frame True {
            w3331 = timestamp(0 s since 1904-01-01)
            n1225 = call <resource>:"UMLEditor getDiagramInfo.vi"("localVariables"=w3341) -> ("graph"=w3327:refnum<class "Graph.lvclass">)  [unwired: 1 in, 17 out]
            n1226 = call-dynamic "getNodes.vi"("reference"=w3327) -> ("nodes"=w3342:refnum<class "AbstractNode.lvclass">[])  [unwired: 16 in, 2 out]
            n1227 = Bundle By Name(cluster=w3324, "LastSync"=w3322) -> (w3323:T5)
            n1228 = for {
              tunnel: w3342 -> [w3375] mode=indexing
              shift-right: [w3370] -> w3339
              shift-left: path[] [] -> [w3371]
              w3374 = refnum<class "ClassNode.lvclass"> refnum  # ClassNode.lvclass
              n1229 = To More Specific Class(target class=w3374, reference=w3375) -> (specific class reference=w3373:refnum<class "ClassNode.lvclass">, error out=w3372:errorcluster)  [unwired: 1 in]
              n1230 = case shown="No Error" w3372 {
                selector: w3372 -> [w3380 _]
                tunnel: w3373 -> [w3381 _]
                tunnel: w3371 -> [w3378 w3386]
                tunnel: [w3377 w3386] -> w3370
                frame No Error {
                  n1231 = call-dynamic "getClassInfo.vi"("reference"=w3381, "error in (no error)"=w3380) -> ("ClassPath"=w3376:path)  [unwired: 8 in, 9 out]
                  n1232 = Empty String/Path?(string/path=w3376) -> (empty?=w3379:bool)
                  n1233 = case shown="True" w3379 {
                    tunnel: w3378 -> [w3384 w3385]
                    tunnel: [w3383 w3385] -> w3377
                    tunnel: w3376 -> [w3382 _]
                    frame False {
                      n1234 = Build Array (concatenate)(w3384, w3382) -> (w3383:path[])
                    }
                    frame True {
                    }
                  }
                }
                frame Error {
                }
              }
            }
            n1235 = for {
              tunnel: w3339 -> [w3358] mode=indexing
              tunnel: path[] [path "Protected/ObjectAttributes.ctl", path "ObjectAttributes.ctl"] -> [w3357]
              shift-right: [w3351] -> w3329
              shift-left: w3331 -> [w3352]
              shift-right: [w3350] -> w3333
              shift-left: w3331 -> [w3348]
              shift-right: [w3345] -> w3332
              shift-left: w3331 -> [w3347]
              n1236 = Strip Path(path=w3358) -> (stripped path=w3356:path)  [unwired: 1 out]
              n1237 = List Folder(path=w3356, pattern="*.vi") -> (path out=w3353:path, filenames=w3355:string[])  [unwired: 2 in, 2 out]
              n1238 = File/Directory Info(path=w3358) -> (last mod=w3346:timestamp)  [unwired: 1 in, 6 out]
              n1239 = for {
                tunnel: w3356 -> [w3369]
                tunnel: w3357 -> [w3368] mode=indexing
                tunnel: [w3365] -> w3349
                stop <- w3366 continue-if-true
                n1240 = Build Path(base path=w3369, name or relative path=w3368) -> (appended path=w3367:path)
                n1241 = File/Directory Info(path=w3367) -> (last mod=w3365:timestamp, error out=w3366:errorcluster)  [unwired: 1 in, 5 out]
              }
              n1242 = for {
                tunnel: w3355 -> [w3363] mode=indexing
                tunnel: w3353 -> [w3364]
                shift-right: [w3359] -> w3351
                shift-left: w3352 -> [w3360]
                n1243 = Build Path(base path=w3364, name or relative path=w3363) -> (appended path=w3362:path)
                n1244 = File/Directory Info(path=w3362) -> (last mod=w3361:timestamp)  [unwired: 1 in, 6 out]
                n1245 = Max & Min(x=w3360, y=w3361) -> (max(x,y)=w3359:timestamp)  [unwired: 1 out]
              }
              n1246 = Max & Min(x=w3348, y=w3349) -> (max(x,y)=w3350:timestamp)  [unwired: 1 out]
              n1247 = Max & Min(x=w3347, y=w3346) -> (max(x,y)=w3345:timestamp)  [unwired: 1 out]
            }
            n1248 = feedback-in #3(w3329) -> ()
            n1249 = feedback #3() -> (w3330:timestamp)  [unwired: 1 in]
            n1250 = feedback-in #4(w3333) -> ()
            n1251 = feedback #4() -> (w3337:timestamp)  [unwired: 1 in]
            n1252 = feedback-in #5(w3332) -> ()
            n1253 = feedback #5() -> (w3338:timestamp)  [unwired: 1 in]
            n1254 = Not Equal?(x=w3329, y=w3330) -> (x != y?=w3328:bool)
            n1255 = Not Equal?(x=w3333, y=w3337) -> (x != y?=w3336:bool)
            n1256 = Not Equal?(x=w3332, y=w3338) -> (x != y?=w3335:bool)
            n1257 = Compound Arithmetic op=OR(w3326, w3328, w3336, w3335) -> (w3325:bool)
            n1258 = case shown="False" w3325 {
              frame False {
                n1259 = Wait (ms)(milliseconds to wait=u32 1000) -> ()  [unwired: 1 out]
                n1260 = local write "StatusBar"("No sync needed, no change was found" ("StatusBar")) -> ()
              }
              frame True {
              }
            }
          }
        }
        n1261 = Bundle By Name(cluster=w3294, "ForceSyncNow"=FALSE ("Sync")) -> (w3306:T5)
        n1262 = Unbundle By Name(w3306) -> ("state"=w3307:T6)
        n1263 = Select(t=UMLEditor_statesType."SyncAll" ("state"), s=w3309, f=w3307) -> (s? t:f=w3311:T6)
      }
      frame "AddNodeFromProjectTree", "AddNodeFromProjectTree+SyncAll" {
        n1264 = call <resource>:"CommonVIs_UmlOpenVIRef.vi"("error in"=w3416) -> ("error out"=w3415:errorcluster, "ProjectNameOut"=w3414:string)  [unwired: 3 in, 6 out]
        n1265 = property on="Picture" class="Pict"() -> ("Mouse"=w3405:T41)  [unwired: 2 in, 2 out]
        n1266 = Unbundle By Name(w3405) -> ("Mouse Position"=w3402:cluster{"X":i32, "Y":i32})
        n1267 = Unbundle By Name(w3401) -> ("zoom"=w3406:dbl, "offset"=w3403:T9)
        n1268 = call <resource>:"GDSProject_GetProjects.vi"("GetProjectRefByName"=w3414, "error in (no error)"=w3415) -> ("Project Refnum"=w3412:refnum<vi>, "error out"=w3413:errorcluster)  [unwired: 1 in, 15 out]
        n1269 = property class="Project"(reference=w3412, error in=w3413) -> (reference out=w3398:refnum<vi>, error out=w3408:errorcluster, "Selected Items in Tree"=w3411:refnum<vi>[], "Window State"=w3387:T53)
        n1270 = Add(x=w3403, y=w3402) -> (x+y=w3404:T9)
        n1271 = Empty Array?(array=w3411) -> (empty?=w3399:bool)
        n1272 = Close Reference(reference=w3398) -> (error out=w3397:errorcluster)  [unwired: 1 in]
        n1273 = Divide(x=w3404, y=w3406) -> (x/y=w3395:T9)
        n1274 = Max & Min(x=w3395, y=T9 {"x"=0.0, "y"=0.0}) -> (max(x,y)=w3393:T9)  [unwired: 1 out]
        n1275 = Unbundle(w3393) -> ("x"=w3392:dbl, "y"=w3391:dbl)
        n1276 = Max & Min(x=w3392, y=w3391) -> (max(x,y)=w3390:dbl)  [unwired: 1 out]
        n1277 = Less?(x=w3390, y=10.0) -> (x < y?=w3388:bool)
        n1278 = Or(x=w3388, y=w3399) -> (x .or. y?=w3400:bool)
        n1279 = case shown="False" w3400 {
          tunnel: w3411 -> [w3432 _]
          tunnel: w3401 -> [w3461 w3582]
          tunnel: [w3460 w3582] -> w3410
          tunnel: [w3457 w3579] -> w3409
          tunnel: w3401 -> [w3419 _]
          tunnel: w3408 -> [w3459 w3580]
          tunnel: [w3458 UMLEditor_statesType."Idle" ("state")] -> w3407
          tunnel: w3393 -> [w3451 _]
          tunnel: w3397 -> [_ _]
          tunnel: w3396 -> [w3428 _]
          tunnel: w3387 -> [_ _]
          frame False {
            # "Node Tool"
            n1280 = call <resource>:"UMLEditor getDiagramInfo.vi"("localVariables"=w3419, "error in (no error)"=w3459) -> ("graph"=w3427:refnum<class "Graph.lvclass">, "diagramType"=w3420:T27, "error out"=w3425:errorcluster)  [unwired: 15 out]
            n1281 = Index Array(array=w3432) -> (element=w3431:refnum<vi>)  [unwired: 1 in]
            n1282 = property class="ProjectItem" props=["Name", "Item ID", "Path", "Reference", "Library Item Type String"](reference=w3431) -> ("Name"=w3455:string, "Item ID"=w3452:string, "Path"=w3453:path, "Reference"=w3450:refnum<vi>)  [unwired: 1 in, 3 out]
            n1283 = call <resource>:"UMLEditor_GetAllClassNodeNames.vi"("error in"=w3425, "graph"=w3427) -> ("error out"=w3424:errorcluster, "ClassNodeNames(WithoutStereotype)"=w3423:string[])  [unwired: 8 out]
            n1284 = Equal?(x=T27 "ClassDiagramGraph" ("diagramType"), y=w3420) -> (x = y?=w3437:bool)
            n1285 = property class="VI"(reference=w3450) -> (reference out=w3439:refnum<vi>, error out=w3449:errorcluster, "Library"=w3448:refnum<vi>)  [unwired: 1 in]
            n1286 = call <vilib>:"Get File Extension.vi"("file"=w3453) -> ("lowercase file extension"=w3434:string)  [unwired: 1 in, 9 out]
            n1287 = Empty String/Path?(string/path=w3434) -> (empty?=w3433:bool)
            n1288 = Not(x=w3433) -> (.not. x?=w3435:bool)
            n1289 = property class="Library"(reference=w3448, error in=w3449) -> (reference out=w3441:refnum<vi>, error out=w3442:errorcluster, "Name"=w3447:string)
            n1290 = Close Reference(reference=w3441, error in (no error)=w3442) -> (error out=w3440:errorcluster)
            n1291 = Close Reference(reference=w3439, error in (no error)=w3440) -> (error out=w3429:errorcluster)
            n1292 = Match Pattern(string=w3455, regular expression="\\.[~\\.]*$") -> (before substring=w3454:string)  [unwired: 4 out]
            n1293 = Match Pattern(string=w3447, regular expression="\\.[~\\.]*$") -> (before substring=w3444:string, offset past match=w3445:i32)  [unwired: 3 out]
            n1294 = case shown="0, Default" w3445 {
              tunnel: w3444 -> [w3567 _]
              tunnel: [w3566 _] -> w3443
              tunnel: w3429 -> [_ _]
              frame 0, Default {
                n1295 = Format Into String(format string="%s : ", w3567) -> (resulting string=w3566:string)  [unwired: 2 in, 1 out]
              }
              frame -1 {
              }
            }
            n1296 = case shown="\"vi\", \"vit\"" w3434 {
              tunnel: w3454 -> [w3569 w3573 w3575]
              tunnel: [w3570 w3574 w3575] -> w3426
              tunnel: w3452 -> [_ _ _]
              tunnel: w3443 -> [_ w3571 _]
              frame "vi", "vit" {
                n1297 = Concatenate Strings("<<VI>>\n" ("string"), w3569) -> (w3570:string)
              }
              frame "ctl", "ctt" {
                n1298 = Concatenate Strings("<<TYPE>>\n" ("string"), w3571, w3573) -> (w3574:string)
              }
              frame Default {
              }
            }
